vi "Read Device Properties.vi"(8 "error in (no error)":errorcluster, 11 "Modbus in":refnum<class "Modbus.lvclass">) -> (0 "error out":errorcluster, 3 "Modbus out":refnum<class "Modbus.lvclass">)   [LabVIEW 2026, in "Modbus.lvlib" / "Modbus.lvclass"]
uses:
  Modbus.lvclass
  C:/Program Files/National Instruments/LabVIEW 2026/vi.lib/FlexLogger/SDK/PluginSDK.lvlibp/PEFClasses/SDK/Plugin/Plugin.lvclass
  <vilib>/FlexLogger/SDK/PluginSDK.lvlibp/PEFClasses/SDK/Processing Element/Timing Parameters.ctl
  <vilib>/FlexLogger/SDK/PluginSDK.lvlibp/PEFClasses/SDK/Processing Element/Timing Method.ctl
  Modbus.lvclass/Modbus.ctl
  Globals/Modbus Strings.vi
  <vilib>/FlexLogger/SDK/PluginSDK.lvlibp/PEFClasses/SDK/Channel/ParameterAccess/Read I32.vi
  <vilib>/FlexLogger/SDK/PluginSDK.lvlibp/PEFClasses/SDK/Channel/ParameterAccess/Read String.vi
  <vilib>/FlexLogger/SDK/PluginSDK.lvlibp/PEFClasses/SDK/Plugin/ParameterAccess/Read Enum.vi
  <vilib>/FlexLogger/SDK/PluginSDK.lvlibp/PEFClasses/SDK/Plugin/ParameterAccess/Read I32.vi
  C:/Program Files/National Instruments/LabVIEW 2026/vi.lib/FlexLogger/SDK/PluginSDK.lvlibp/PEFClasses/SDK/Processing Element/Processing Element.lvclass
  D:/Work/FlexLogger/Features/Modbus Plugin/Modbus - Working Copy/Modbus/Modbus.lvclass
  <vilib>/FlexLogger/SDK/PluginSDK.lvlibp/PEFClasses/SDK/Plugin/Plugin.lvclass
  <vilib>/FlexLogger/SDK/PluginSDK.lvlibp/PEFClasses/SDK/Channel/Channel.lvclass
  <vilib>/FlexLogger/SDK/PluginSDK.lvlibp/PEFClasses/SDK/Processing Element/Processing Element.lvclass
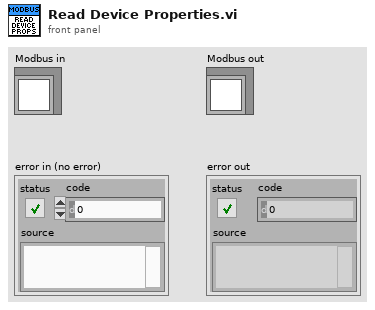
[diagram p1: front panel]
types:
  T1 = typedef "PluginSDK.lvlibp/Processing Element.lvclass/Timing Parameters.ctl" = cluster{"Timing Method":T2, "Timing Period (ms)":i32}
  T2 = typedef "PluginSDK.lvlibp/Processing Element.lvclass/Timing Method.ctl" = enum16{"Periodic", "Immediate", "On Data Ready", "Triggered"}
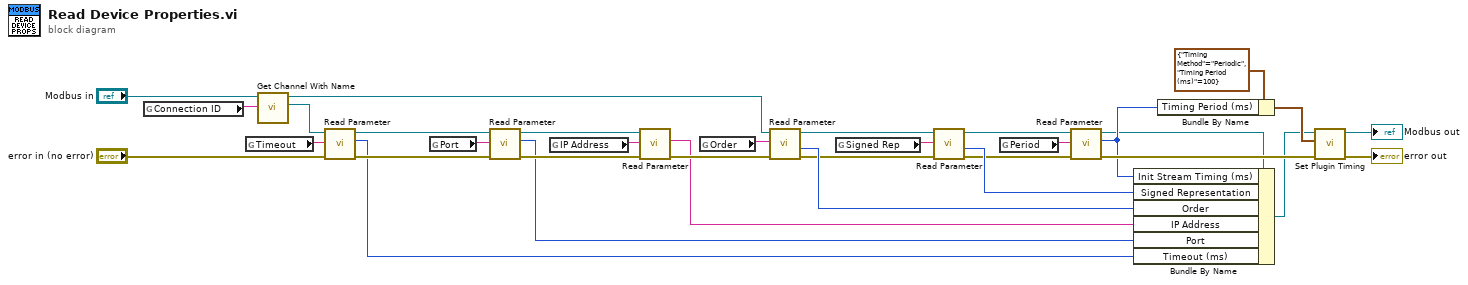
[diagram p0: block diagram]
diagram:
  n1 = global read "Modbus Strings.vi" "Connection ID"() -> (w33:string)
  n2 = global read "Modbus Strings.vi" "Timeout"() -> (w32:string)
  n3 = call <vilib>:"Get Channel With Name.vi"("Name"=w33, "Plugin in"="Modbus in") -> ("Channel"=w25:refnum<class "Channel.lvclass">, "Plugin out"=w13:refnum<class "Modbus.lvclass">)  [unwired: 7 in, 1 out]
  n4 = call-poly <vilib>:"Read Parameter.vi"("error in (no error)"="error in (no error)", "Name"=w32, "Channel in"=w25) -> ("error out"=w26:errorcluster, "Value"=w24:i32, "Channel out"=w27:refnum<class "Channel.lvclass">)  [unwired: 5 in, 1 out]
  n5 = global read "Modbus Strings.vi" "Port"() -> (w28:string)
  n6 = call-poly <vilib>:"Read Parameter.vi"("error in (no error)"=w26, "Name"=w28, "Channel in"=w27) -> ("error out"=w30:errorcluster, "Value"=w20:i32, "Channel out"=w31:refnum<class "Channel.lvclass">)  [unwired: 5 in, 1 out]
  n7 = global read "Modbus Strings.vi" "IP Address"() -> (w29:string)
  n8 = call-poly <vilib>:"Read Parameter.vi"("error in (no error)"=w30, "Name"=w29, "Channel in"=w31) -> ("error out"=w14:errorcluster, "Value"=w12:string)  [unwired: 5 in, 2 out]
  n9 = global read "Modbus Strings.vi" "Order"() -> (w15:string)
  n10 = call-poly <vilib>:"Read Parameter.vi"("error in (no error)"=w14, "Name"=w15, "Plugin in"=w13) -> ("error out"=w17:errorcluster, "Index"=w19:i32, "Plugin out"=w16:refnum<class "Modbus.lvclass">)  [unwired: 4 in, 2 out]
  n11 = global read "Modbus Strings.vi" "Signed Rep"() -> (w18:string)
  n12 = call-poly <vilib>:"Read Parameter.vi"("error in (no error)"=w17, "Name"=w18, "Plugin in"=w16) -> ("error out"=w6:errorcluster, "Index"=w21:i32, "Plugin out"=w7:refnum<class "Modbus.lvclass">)  [unwired: 4 in, 2 out]
  n13 = global read "Modbus Strings.vi" "Period"() -> (w11:string)
  n14 = call-poly <vilib>:"Read Parameter.vi"("error in (no error)"=w6, "Name"=w11, "Plugin in"=w7) -> ("error out"=w10:errorcluster, "Value"=w5:i32, "Plugin out"=w4:refnum<class "Modbus.lvclass">)  [unwired: 5 in, 1 out]
  n15 = Bundle By Name(cluster=w4, "Init Stream Timing (ms)"=w5, "Signed Representation"=w21, "Order"=w19, "IP Address"=w12, "Port"=w20, "Timeout (ms)"=w24) -> (w3:refnum<class "Modbus.lvclass">)
  n16 = Bundle By Name(cluster=T1 {"Timing Method"=enum."Periodic", "Timing Period (ms)"=100} ("Timing Parameters"), "Timing Period (ms)"=w5) -> (w9:T1)
  n17 = call <vilib>:"Set Plugin Timing.vi"("error in (no error)"=w10, "Timing Parameters"=w9, "Plugin in"=w3) -> ("error out"=→"error out":errorcluster, "Plugin out"=→"Modbus out":refnum<class "Modbus.lvclass">)  [unwired: 7 in]
